vi "Find Tagged and Move.vi"(6 "position":T1, 7 "TagName":string="phygbuTag", 8 "error in":errorcluster, 9 "TagValue":string, 10 "Destination Diagram":refnum<vi>, 11 "VI Refnum":refnum<vi>) -> (0 "error out":errorcluster, 3 "Moved Tagged object":refnum<vi>)   [LabVIEW 2012, in "Scripting Tools.lvlib"]
doc: "Find a node with the given tag and value in the Vi referenced and move it to the block diagram given by the diagram reference"
uses:
  Scripting Tools.lvlib
  <vilib>/Utility/miscctls.llb/LVPositionTypeDef.ctl
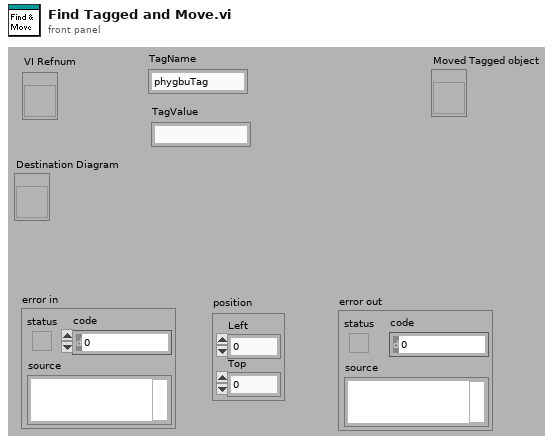
[diagram p1: front panel]
types:
  T1 = typedef "LVPositionTypeDef.ctl" = cluster{"Left":i32, "Top":i32}
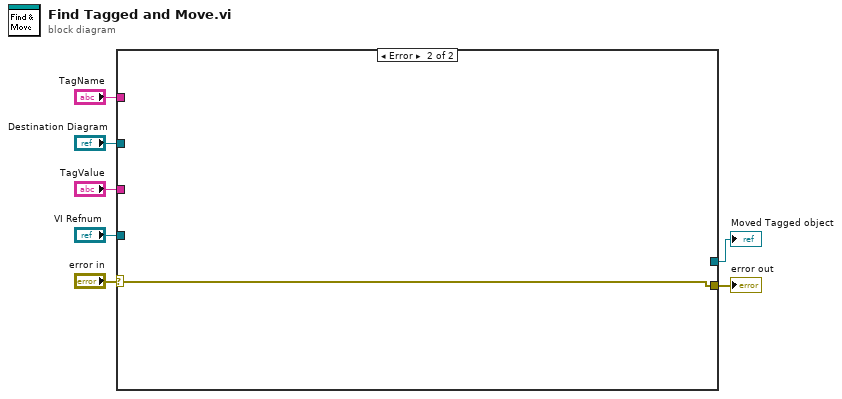
[diagram p0: block diagram]
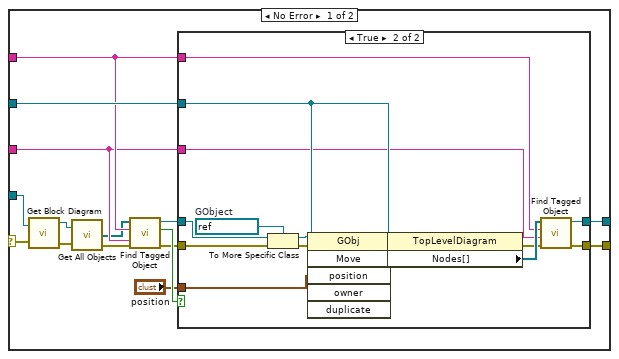
[diagram p2: hidden frame]
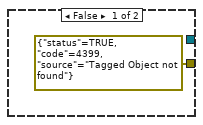
[diagram p3: hidden frame]
diagram:
  n1 = case shown="Error" "error in" {
    selector: "error in" -> [w8 w38]
    tunnel: "VI Refnum" -> [w22 _]
    tunnel: "Destination Diagram" -> [w18 _]
    tunnel: "TagName" -> [w16 _]
    tunnel: "TagValue" -> [w15 _]
    tunnel: [w14 _] -> w3
    tunnel: [w9 w38] -> w2
    frame No Error {
      n2 = call "Get Block Diagram.vi"("vi refnum in"=w22, "error in (no error)"=w8) -> ("Diagram"=w13:refnum<vi>, "error out"=w12:errorcluster)  [unwired: 1 out]
      n3 = call "Get All Objects.vi"("Diagram In"=w13, "error in"=w12) -> ("All Objects"=w10:refnum<vi>[], "error out"=w11:errorcluster)  [unwired: 1 out]
      n4 = call "Find Tagged Object.vi"("error in (no error)"=w11, "TagValue"=w15, "TagName"=w16, "Array of References"=w10) -> ("error out"=w20:errorcluster, "Found?"=w21:bool, "reference"=w19:refnum<vi>)  [unwired: 1 in, 4 out]
      n5 = case shown="True" w21 {
        tunnel: w20 -> [_ w36]
        tunnel: w19 -> [_ w37]
        tunnel: w18 -> [_ w30]
        tunnel: "position" -> [_ w32]
        tunnel: w16 -> [_ w28]
        tunnel: w15 -> [_ w27]
        tunnel: [_ w25] -> w14
        tunnel: [errorcluster {"status"=TRUE, "code"=4399, "source"="Tagged Object not found"} ("error out") w24] -> w9
        frame False {
        }
        frame True {
          w35 = refnum<vi> refnum  # GObject
          n6 = To More Specific Class(target class=w35, reference=w37, error in=w36) -> (specific class reference=w34:refnum<vi>, error out=w33:errorcluster)
          n7 = invoke class="GObj" method="Move"(reference=w34, error in=w33, "position"=w32, "owner"=w30) -> (error out=w31:errorcluster)  [unwired: 2 in, 5 out]
          n8 = property on="Property Node" class="TopLevelDiagram"(reference=w30, error in=w31) -> (error out=w26:errorcluster, "Nodes[]"=w29:refnum<vi>[])  [unwired: 1 out]
          n9 = call "Find Tagged Object.vi"("error in (no error)"=w26, "TagValue"=w27, "TagName"=w28, "Array of References"=w29) -> ("error out"=w24:errorcluster, "reference"=w25:refnum<vi>)  [unwired: 1 in, 5 out]
        }
      }
    }
    frame Error {
    }
  }
  "Moved Tagged object" <- w3
  "error out" <- w2
